vi "Run greeter_server.vi"() -> ()   [LabVIEW 2019, in "helloworld_server.lvlib"]
uses:
  helloworld_server.lvlib
  RPC Service/Greeter/Greeter.lvclass
  C:/Program Files (x86)/National Instruments/LabVIEW 2019/vi.lib/gRPC/LabVIEW gRPC Servicer/ServiceBase/ServiceBase.lvclass
  <vilib>/gRPC/LabVIEW gRPC Servicer/Servicer/Servicer.lvclass/Servicer.ctl
  <vilib>/gRPC/LabVIEW gRPC Servicer/Servicer/Servicer.lvclass
panel:
  in  "error in":errorcluster
  out "error out":errorcluster
  out "Listening Port":i32
  in  "Stop":bool
  in  "Server Address":string="localhost:50051"
  in  "Server Certificate File (.crt)":path
  in  "Server Key File (.key)":path
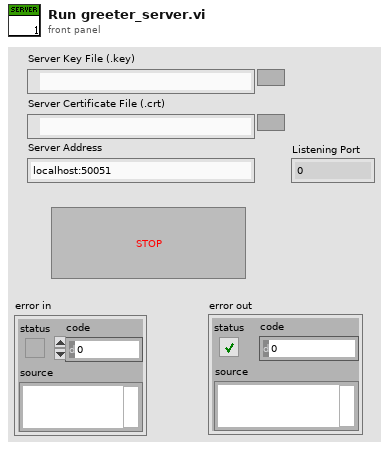
[diagram p1: front panel]
types:
  T1 = typedef "grpc-lvsupport-release.lvlib/grpcId.ctl" = u64
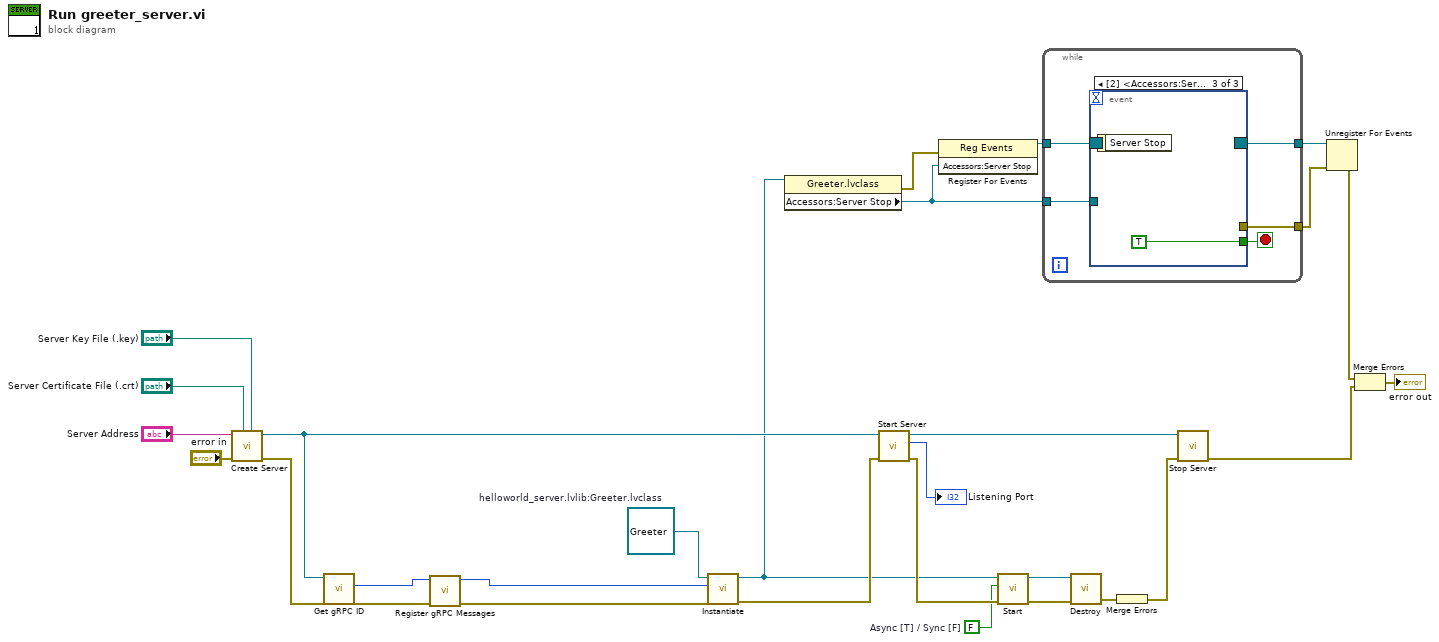
[diagram p0: block diagram]
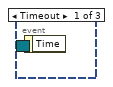
[diagram p2: hidden frame]
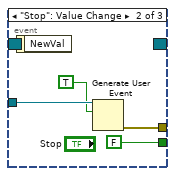
[diagram p3: hidden frame]
diagram:
  w8 = FALSE  # Async [T] / Sync [F]
  w5 = refnum<class "Greeter.lvclass"> refnum  # helloworld_server.lvlib:Greeter.lvclass
  n1 = call <vilib>:"Create Server.vi"("Server Key File (.key)"="Server Key File (.key)", "Server Certificate File (.crt)"="Server Certificate File (.crt)", "error in"="error in", "Server Address"="Server Address") -> ("error out"=w14:errorcluster, "gRPC Server out"=w21:refnum<class "Servicer.lvclass">)  [unwired: 6 in]
  n2 = call <vilib>:"Get gRPC ID.vi"("OOP Server in"=w21) -> ("gRPC ID"=w15:T1)  [unwired: 9 in, 1 out]
  n3 = call "Register gRPC Messages.vi"("error in (no error)"=w14, "gRPC ID"=w15) -> ("error out"=w13:errorcluster, "gRPC ID Out"=w12:T1)  [unwired: 8 in]
  n4 = call-dynamic "Instantiate.vi"("error in"=w13, "gRPCid"=w12, "iService"=w5) -> ("error out"=w19:errorcluster, "iService"=w7:refnum<class "Greeter.lvclass">)  [unwired: 7 in]
  n5 = property class="Greeter.lvclass"(reference=w7) -> (error out=w20:errorcluster, "Accessors:Server Stop"=w6:refnum<user-event>)  [unwired: 1 in, 1 out]
  n6 = call <vilib>:"Start Server.vi"("error in"=w19, "gRPC Server in"=w21) -> ("error out"=w11:errorcluster, "Listening Port"=→"Listening Port":i32, "gRPC Server out"=w28:refnum<class "Servicer.lvclass">)  [unwired: 7 in]
  n7 = register-events(error in=w20, w6) -> (reference out=w24:refnum<event-registration>)  [unwired: 1 in, 1 out]
  n8 = call-dynamic "Start.vi"("error in"=w11, "ASync [T]"=w8, "iService in"=w7) -> ("error out"=w10:errorcluster, "iService out"=w9:refnum<class "Greeter.lvclass">)  [unwired: 7 in]
  n9 = while {
    tunnel: w24 -> [w33]
    tunnel: [w31] -> w23
    tunnel: [w29] -> w16
    tunnel: w6 -> [w30]
    stop <- w32 stop-if-true
    n10 = event shown="[2] <Accessors:Server Stop>: User Event" {
      selector: w33 -> [_ _ _]
      dyn-events: [_ _ _] -> w31
      timeout: _ -> [_ _ _]
      tunnel: [_ FALSE TRUE] -> w32
      tunnel: w30 -> [_ w36 _]
      tunnel: [_ w34 _] -> w29
      event Timeout {
        n11 = event-data() -> ()  [unwired: 1 in, 1 out]
      }
      event "Stop": Value Change {
        n12 = event-data() -> ()  [unwired: 1 in, 1 out]
        n13 = Generate User Event(user event=w36, event data cluster=TRUE ("event data")) -> (error out=w34:errorcluster)  [unwired: 2 in, 1 out]
      }
      event User Event {
        n14 = event-data() -> ()  [unwired: 1 in, 1 out]
      }
    }
  }
  n15 = call-dynamic "Destroy.vi"("error in (no error)"=w10, "SignalGeneratorService in"=w9) -> ("error out"=w18:errorcluster)  [unwired: 8 in, 1 out]
  n16 = Merge Errors(w18) -> (w17:errorcluster)
  n17 = call <vilib>:"Stop Server.vi"("error in"=w17, "gRPC Server in"=w28) -> ("error out"=w4:errorcluster)  [unwired: 9 in]
  n18 = Unregister For Events(event registration refnum=w23, error in=w16) -> (error out=w3:errorcluster)
  n19 = Merge Errors(w3, w4) -> (→"error out":errorcluster)
